vi "Write CLI Reference.vi"(8 "error in":errorcluster, 10 "CLI":refnum<class "CLI.lvclass">, 11 "Console Logger in":refnum<class "Console Logger.lvclass">) -> (0 "error out":errorcluster, 3 "Console Logger out":refnum<class "Console Logger.lvclass">)   [LabVIEW 2026, in "Console Logger.lvlib" / "Console Logger.lvclass"]
doc: "Data accessor."
uses:
  Console Logger.lvclass
  <vilib>/Wiresmith Technology/G CLI/CLI Class/CLI.lvclass
  Console Logger.lvclass/Console Logger.ctl
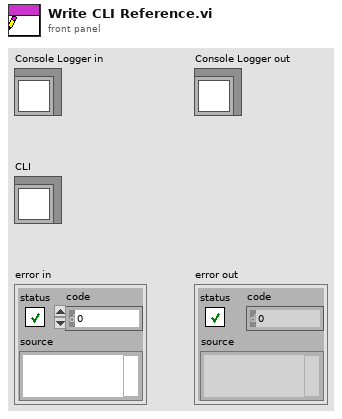
[diagram p1: front panel]
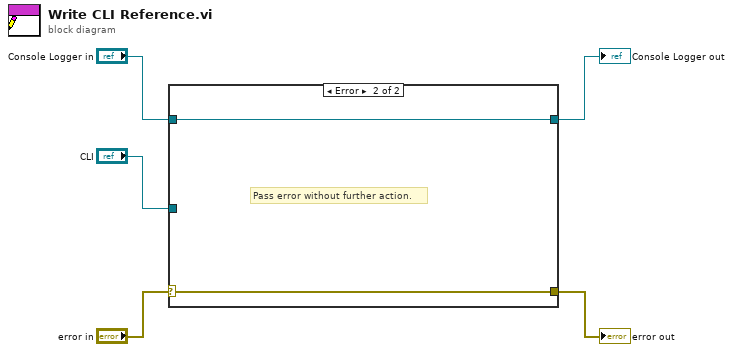
[diagram p0: block diagram]
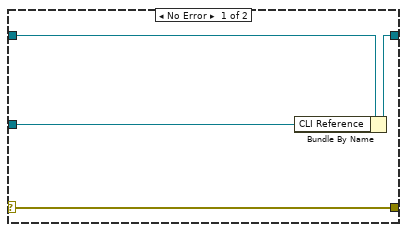
[diagram p2: hidden frame]
diagram:
  n1 = case shown="Error" "error in" {
    selector: "error in" -> [w9 w11]
    tunnel: [w9 w11] -> w4
    tunnel: [w7 w10] -> w2
    tunnel: "Console Logger in" -> [w8 w10]
    tunnel: "CLI" -> [w6 _]
    frame No Error {
      n2 = Bundle By Name(cluster=w8, "CLI Reference"=w6) -> (w7:refnum<class "Console Logger.lvclass">)
    }
    frame Error {
      # "Pass error without further action."
    }
  }
  "error out" <- w4
  "Console Logger out" <- w2
